vi "set next wppos.vi"(8 "error in (no error)":errorcluster, 11 "S4ICS in":refnum<class "S4ICS.lvclass">) -> (0 "error out":errorcluster, 3 "S4ICS out":refnum<class "S4ICS.lvclass">)   [LabVIEW 2018, in "S4ICS.lvclass"]
uses:
  S4ICS.lvclass
  S4ICS.lvclass/S4ICS.ctl
  Mechanism/Mechanism.lvclass
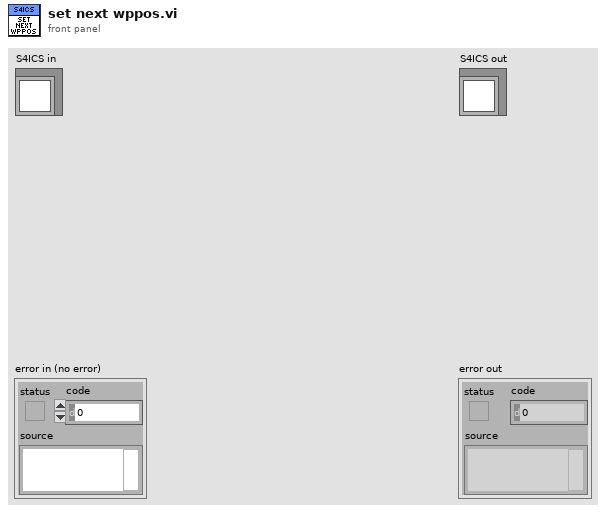
[diagram p1: front panel]
types:
  T1 = cluster{"mode":string, "condition":string, "position":string, "pos_name":string, "pos_id":string}
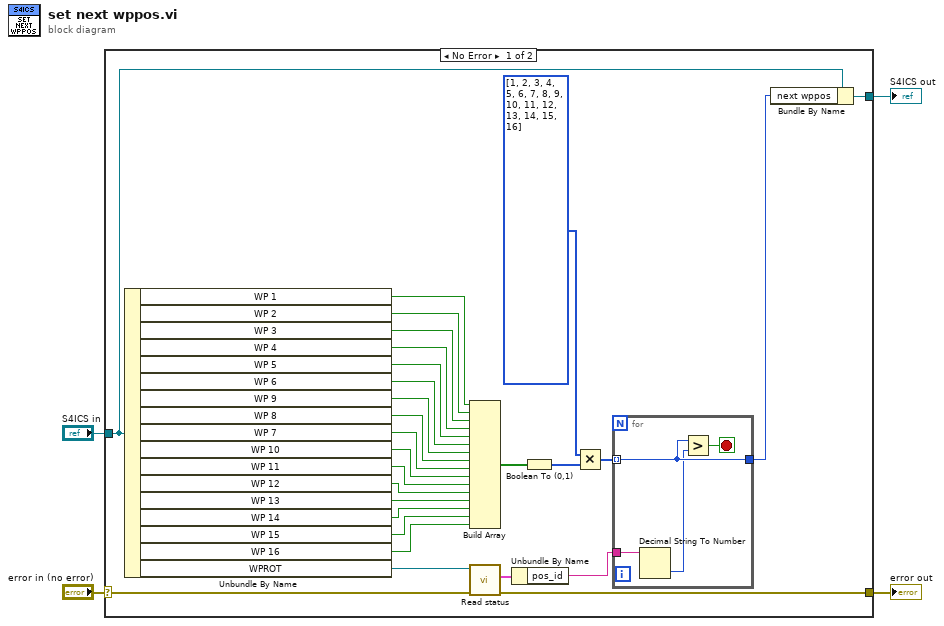
[diagram p0: block diagram]
diagram:
  n1 = case shown="No Error" "error in (no error)" {
    selector: "error in (no error)" -> [w30 w38]
    tunnel: [w10 w38] -> w3
    tunnel: [w6 w37] -> w1
    tunnel: "S4ICS in" -> [w7 w37]
    frame No Error {
      n2 = Unbundle By Name(w7) -> ("WP 1"=w29:bool, "WP 2"=w28:bool, "WP 3"=w27:bool, "WP 4"=w26:bool, "WP 5"=w25:bool, "WP 6"=w24:bool, "WP 9"=w23:bool, "WP 8"=w22:bool, "WP 7"=w21:bool, "WP 10"=w20:bool, "WP 11"=w19:bool, "WP 12"=w18:bool, "WP 13"=w17:bool, "WP 14"=w16:bool, "WP 15"=w15:bool, "WP 16"=w14:bool, "WPROT"=w31:refnum<class "Mechanism.lvclass">)
      n3 = Build Array(w29, w28, w27, w26, w25, w24, w23, w22, w21, w20, w19, w18, w17, w16, w15, w14) -> (w13:bool[])
      n4 = call-dynamic "Read status.vi"("error in (no error)"=w30, "Mechanism in"=w31) -> ("error out"=w10:errorcluster, "status"=w32:T1)  [unwired: 7 in, 1 out]
      n5 = Unbundle By Name(w32) -> ("pos_id"=w8:string)
      n6 = Boolean To (0,1)(Boolean=w13) -> (0, 1=w12:i16[])
      n7 = Multiply(x=i32[] [1, 2, 3, 4, 5, 6, 7, 8, 9, 10, 11, 12, 13, 14, 15, 16], y=w12) -> (x*y=w9:i32[])
      n8 = for {
        tunnel: w9 -> [w35] mode=indexing
        tunnel: w8 -> [w34]
        tunnel: [w35] -> w5
        stop <- w36 stop-if-true
        n9 = Decimal String To Number(string=w34) -> (number=w33:i32)  [unwired: 2 in, 1 out]
        n10 = Greater?(x=w35, y=w33) -> (0:w36:bool)
      }
      n11 = Bundle By Name(cluster=w7, "next wppos"=w5) -> (w6:refnum<class "S4ICS.lvclass">)
    }
    frame Error {
    }
  }
  "error out" <- w3
  "S4ICS out" <- w1
